vi "Toolbar Faacade.vi"(0 "Data In":T5, 2 "Display State In":T2={"Buttons Displayed"=0, "Button States"=[], "Button Size"=0, "Button Style"=enum."Classic", "Active Button"=0, "Force Regen?"=FALSE, "Tip String Ref"=refnum}, 3 "Container State":T4) -> (6 "Data Out":T5, 7 "Display State Out":T2={"Buttons Displayed"=0, "Button States"=[], "Button Size"=0, "Button Style"=enum."Classic", "Active Button"=0, "Force Regen?"=FALSE, "Tip String Ref"=refnum}, 8 "Action":T1)   [LabVIEW 2012, in "Toolbar.xctl"]
doc: "The business end of the XControl..."
uses:
  Toolbar.xctl
  Toolbar Data.ctl
  Button_Class/Type Defs/Button Events.ctl
  <vilib>/_xctls/Container State.ctl
  Toolbar State.ctl
  Button_Class/Button.lvclass
  Button_Class/Type Defs/Button Style.ctl
  <vilib>/_xctls/Action.ctl
  Button_Class/Type Defs/Button Status.ctl
  <vilib>/_xctls/XControlSupport.lvlib
panel:
  out "Display":picture[](array[picture])
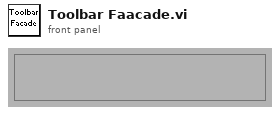
[diagram p1: front panel]
types:
  T1 = typedef "XControlSupport.lvlib/Action.ctl" = cluster{"Data Changed?":bool, "State Changed?":bool, "Action Name":string}
  T2 = typedef "Toolbar.xctl/Toolbar State.ctl" = cluster{"Buttons Displayed":i32, "Button States":refnum<class "Button.lvclass">[], "Button Size":i32, "Button Style":T3, "Active Button":i32, "Force Regen?":bool, "Tip String Ref":refnum<vi>}
  T3 = typedef "Button.lvclass/Button Style.ctl" = enum16{"System", "Modern", "Classic", "Rounded", "Silver", "Ni Theme", "Metallic"}
  T4 = typedef "XControlSupport.lvlib/Container State.ctl" = cluster{"Indicator?":bool, "Run Mode?":bool, " Refnum":refnum<vi>}
  T5 = typedef "Toolbar.xctl/Toolbar Data.ctl" = cluster{"Index":i32, "Type":T6}
  T6 = typedef "Button.lvclass/Button Events.ctl" = enum16{"Click", "Latch", "Unlatch"}
  T7 = enum16{"NoButton", "Left Button", "Right Button", "Middle Button"}
  T8 = typedef "Button.lvclass/Button Status.ctl" = enum16{"Off", "Hover", "On", "Disabled"}
  T9 = typedef "LVPoint32TypeDef.ctl" = cluster{"Horizontal":i32, "Vertical":i32}
  T10 = typedef "LVRectTypeDef.ctl" = cluster{"Left":i16, "Top":i16, "Right":i16, "Bottom":i16}
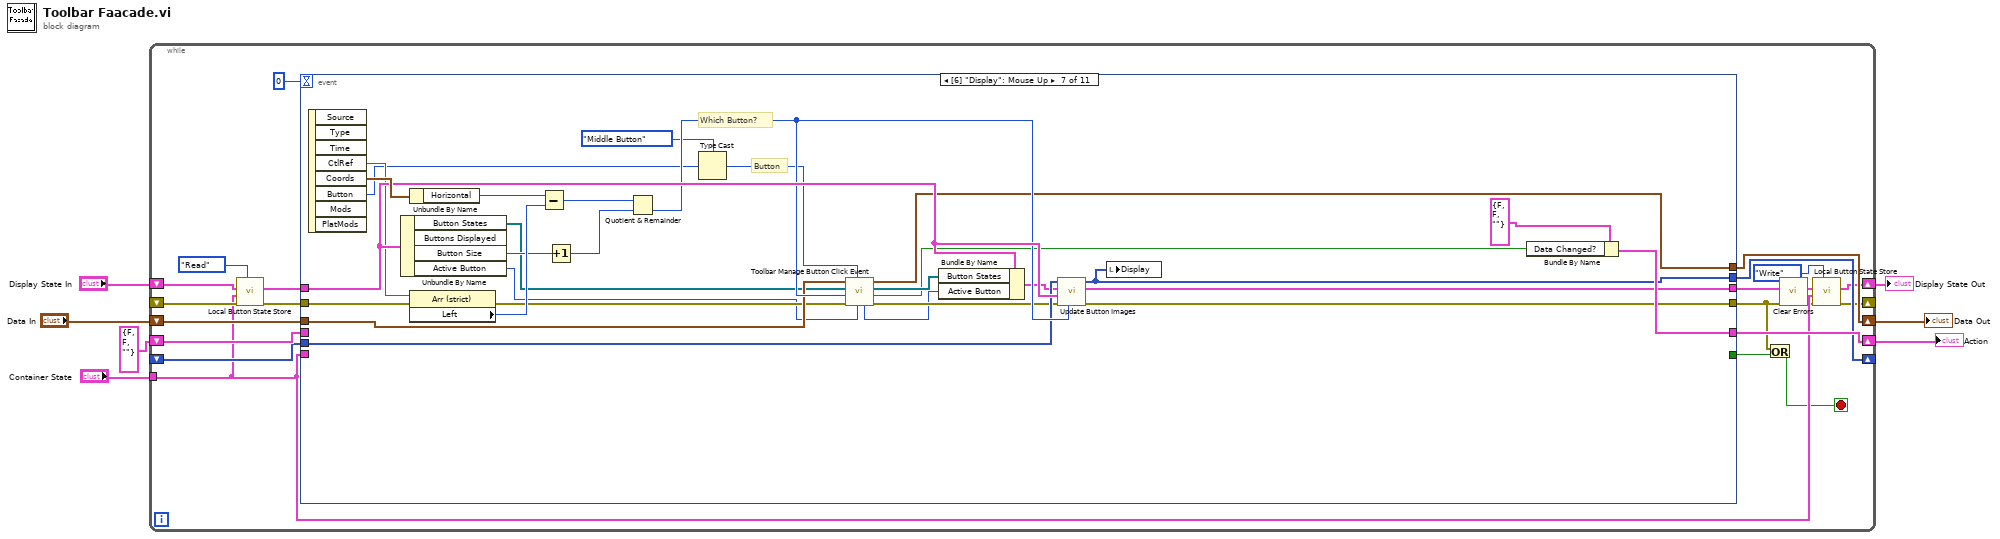
[diagram p0: block diagram]
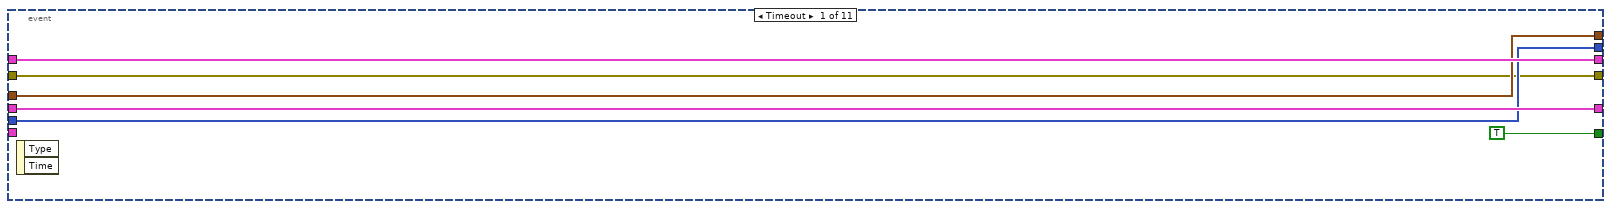
[diagram p2: hidden frame]
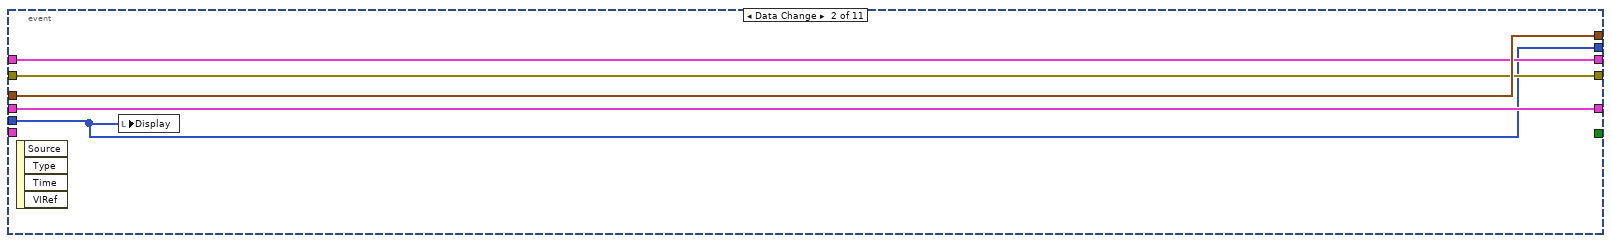
[diagram p3: hidden frame]
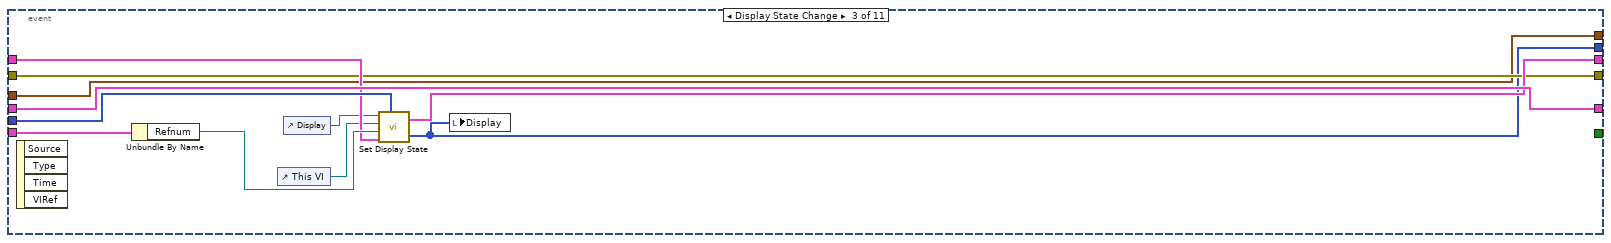
[diagram p4: hidden frame]
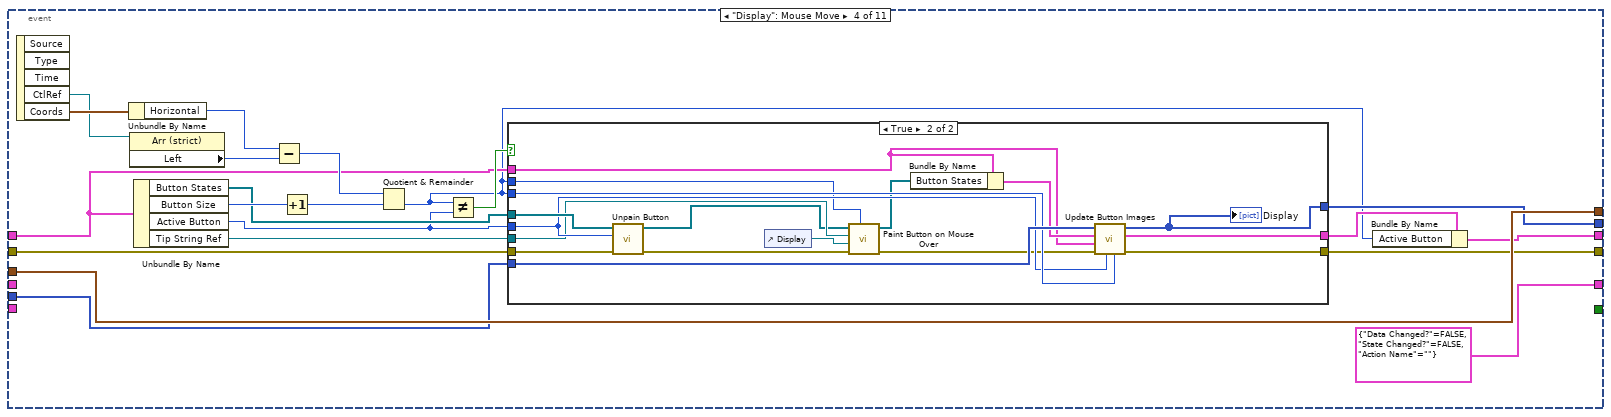
[diagram p5: hidden frame]
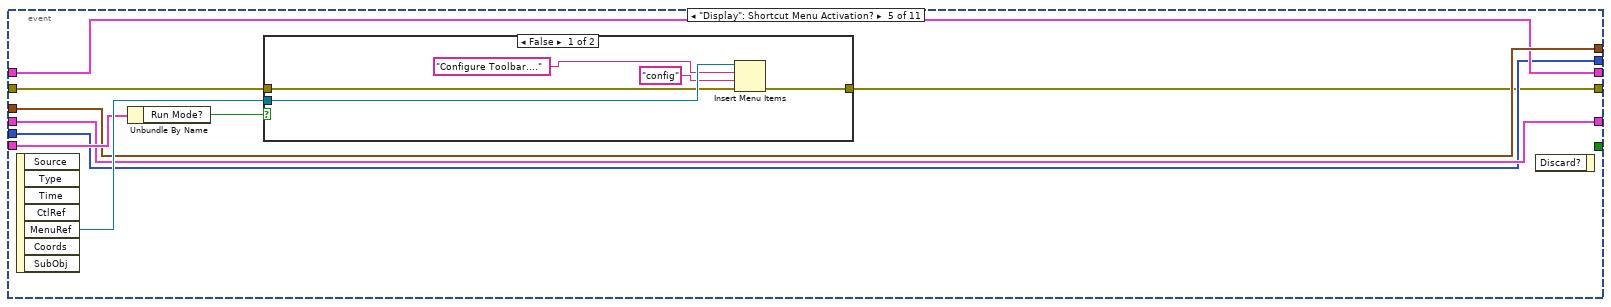
[diagram p7: hidden frame]
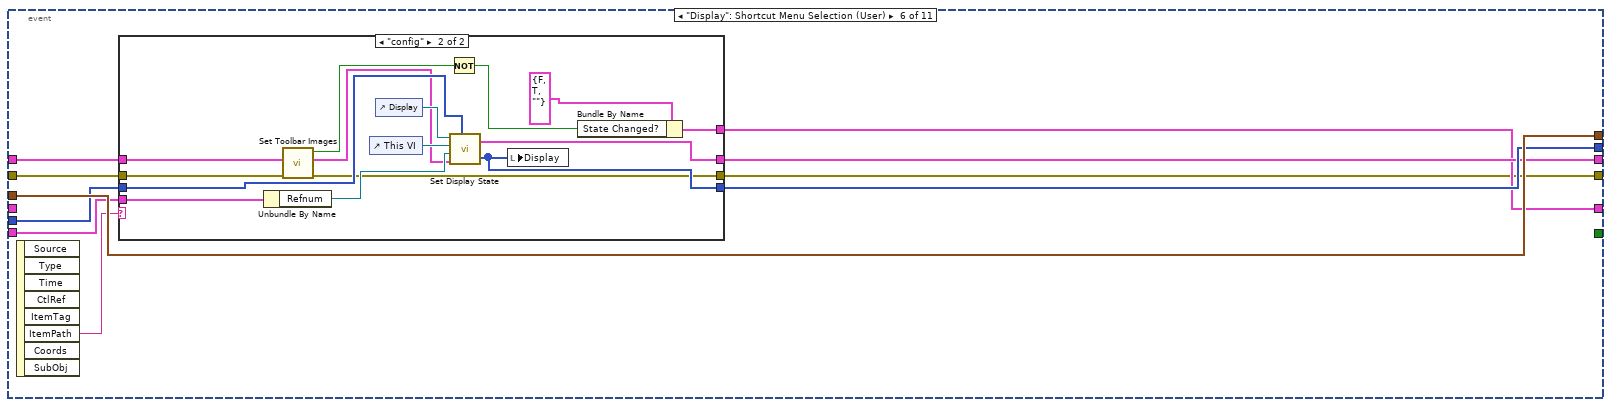
[diagram p9: hidden frame]
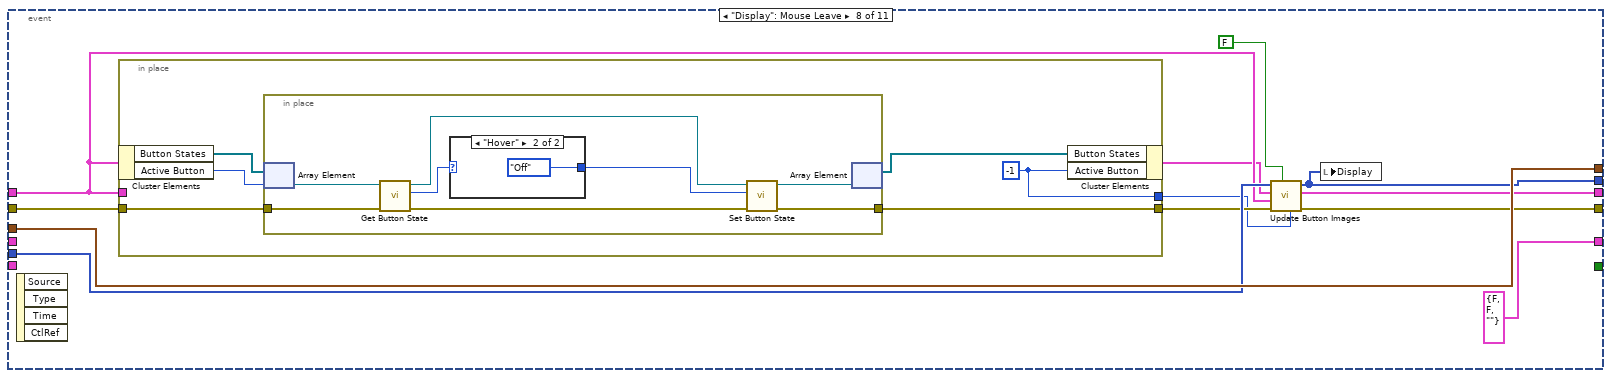
[diagram p11: hidden frame]
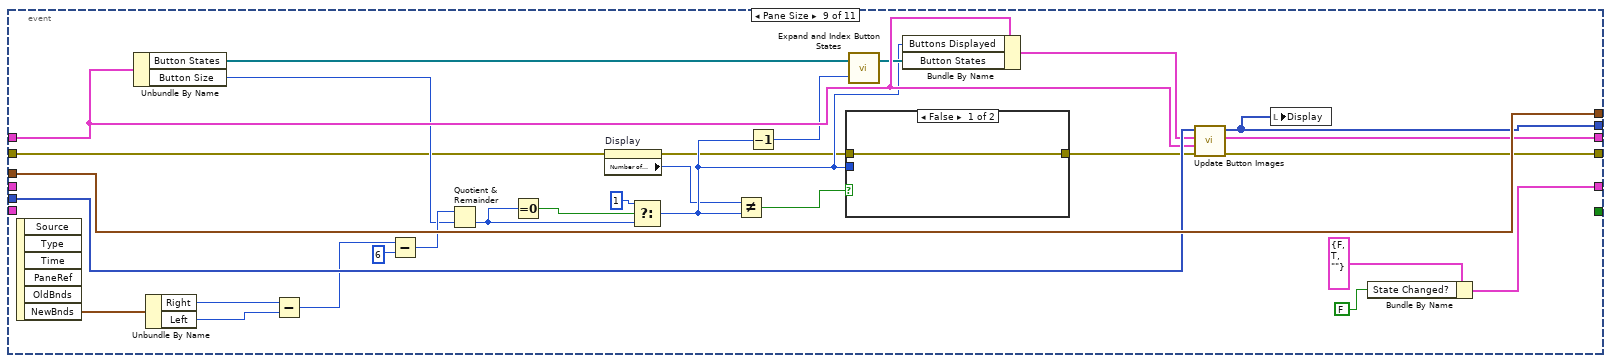
[diagram p13: hidden frame]
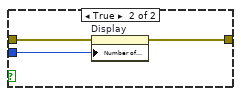
[diagram p14: hidden frame]
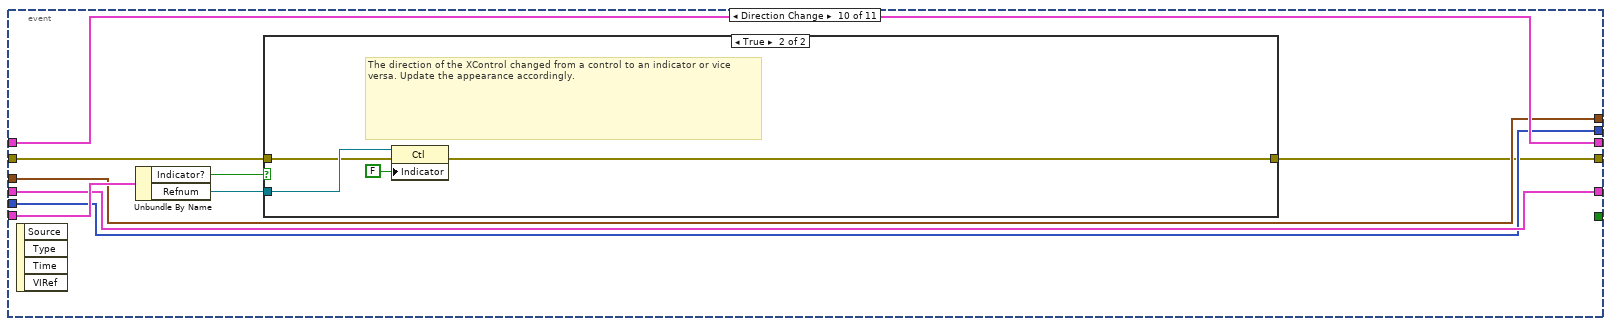
[diagram p15: hidden frame]
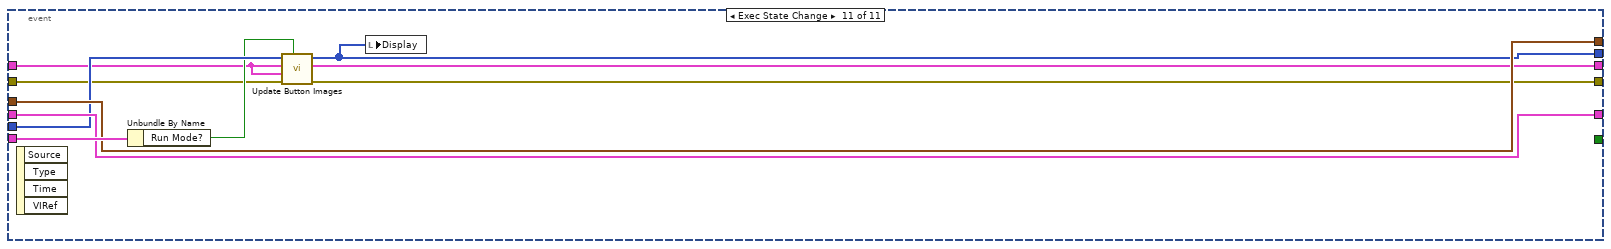
[diagram p17: hidden frame]
diagram:
  n1 = while {
    shift-right: [w11] -> w4
    shift-left: "Display State In" -> [w15]
    tunnel: "Container State" -> [w13]
    shift-right: [w25] -> w7
    shift-left: "Data In" -> [w26]
    shift-right: [w23] -> w2
    shift-left: T1 {"Data Changed?"=FALSE, "State Changed?"=FALSE, "Action Name"=""} ("Action") -> [w24]
    shift-right: [w22] -> _
    shift-left: _ -> [w21]
    shift-right: [w18] -> _
    shift-left: _ -> [w17]
    stop <- w10 stop-if-true
    n2 = call "Local Button State Store.vi"("Operation"=enum16{"Read", "Write"}."Read", "error in (no error)"=w17, "Container State"=w13, "Display State In"=w15) -> ("error out"=w16:errorcluster, "Display State Out"=w12:T2)  [unwired: 6 out]
    n3 = event shown="[6] \"Display\": Mouse Up" {
      selector: _ -> [_ _ _ _ _ _ _ _ _ _ _]
      dyn-events: _ -> [_ _ _ _ _ _ _ _ _ _ _]
      timeout: 0 -> [_ _ _ _ _ _ _ _ _ _ _]
      tunnel: w12 -> [w32 w38 w46 w55 w96 w115 w160 w167 w209 w232 w242]
      tunnel: [w32 w38 w43 w54 w96 w112 w155 w172 w207 w232 w241] -> w14
      tunnel: [TRUE _ _ _ _ _ _ _ _ _ _] -> w28
      tunnel: w13 -> [_ _ w48 _ w99 w111 _ _ _ w233 w248]
      tunnel: w26 -> [w31 w39 w41 w68 w97 w116 w153 w174 w215 w231 w247]
      tunnel: [w31 w39 w41 w68 w97 w116 w152 w174 w215 w231 w247] -> w25
      tunnel: [w33 w37 w50 T1 {"Data Changed?"=FALSE, "State Changed?"=FALSE, "Action Name"=""} ("Action") w95 w110 w163 T1 {"Data Changed?"=FALSE, "State Changed?"=FALSE, "Action Name"=""} ("Action") w200 w230 w246] -> w23
      tunnel: w24 -> [w33 w37 w50 _ w95 _ _ _ _ w230 w246]
      tunnel: [w30 w35 w40 w64 w94 w113 w151 w164 w193 w229 w244] -> w22
      tunnel: w21 -> [w30 w35 w49 w63 w94 w114 w150 w173 w213 w229 w245]
      tunnel: [w29 w36 w42 w59 w93 w108 w145 w169 w197 w225 w239] -> w9
      tunnel: w16 -> [w29 w36 w42 w58 w92 w109 w144 w171 w194 w226 w240]
      event Timeout {
        n4 = event-data() -> ()  [unwired: 3 out]
      }
      event Data Change {
        n5 = event-data() -> ()  [unwired: 5 out]
        n6 = local write "Display"(w35) -> ()
      }
      event Display State Change {
        n7 = event-data() -> ()  [unwired: 5 out]
        n8 = Unbundle By Name(w48) -> ("Refnum"=w47:refnum<vi>)
        n9 = control-ref of="This VI"() -> (w45:refnum<vi>)
        n10 = control-ref of="Display"() -> (w44:refnum<vi>)
        n11 = call "Set Display State.vi"("Picture Array Refnum"=w44, "Facade Vi Refnum"=w45, "Container Refnum"=w47, "Display State In"=w46, "Display"=w49) -> ("State Out"=w43:T2, "Images Out"=w40:picture[])
        n12 = local write "Display"(w40) -> ()
      }
      event "Display": Mouse Move {
        n13 = event-data() -> ("CtlRef"=w67:refnum<vi>, "Coords"=w70:T9)  [unwired: 4 out]
        n14 = Unbundle By Name(w70) -> ("Horizontal"=w69:i32)
        n15 = property class="Arr (strict)"(reference=w67) -> ("Left"=w65:i32)  [unwired: 1 in, 2 out]
        n16 = Unbundle By Name(w55) -> ("Button States"=w57:refnum<class "Button.lvclass">[], "Button Size"=w61:i32, "Active Button"=w52:i32, "Tip String Ref"=w51:refnum<vi>)
        n17 = Subtract(x=w69, y=w65) -> (x-y=w66:i32)
        n18 = Increment(x=w61) -> (x+1=w60:i32)
        n19 = Quotient & Remainder(x=w66, y=w60) -> (floor(x/y)=w53:i32)  [unwired: 1 out]
        n20 = Not Equal?(x=w53, y=w52) -> (x != y?=w56:bool)
        n21 = case shown="True" w56 {
          tunnel: [w74 w80] -> w64
          tunnel: w63 -> [w74 w91]
          tunnel: w55 -> [w73 w79]
          tunnel: [w73 w89] -> w62
          tunnel: [w72 w75] -> w59
          tunnel: w58 -> [w72 w85]
          tunnel: w57 -> [_ w87]
          tunnel: w53 -> [_ w84]
          tunnel: w52 -> [_ w86]
          tunnel: w53 -> [_ w88]
          tunnel: w51 -> [_ w78]
          frame False {
          }
          frame True {
            n22 = call "Unpain Button.vi"("error in (no error)"=w85, "Old Button"=w86, "Button States in"=w87) -> ("error out"=w83:errorcluster, "Button States out"=w77:refnum<class "Button.lvclass">[])  [unwired: 7 in]
            n23 = control-ref of="Display"() -> (w76:refnum<vi>)
            n24 = call "Paint Button on Mouse Over.vi"("New Active Button"=w84, "error in (no error)"=w83, "Array in"=w76, "Tip String Ref"=w78, "Button States in"=w77) -> ("error out"=w81:errorcluster, "Button States out"=w82:refnum<class "Button.lvclass">[])  [unwired: 5 in]
            n25 = Bundle By Name(cluster=w79, "Button States"=w82) -> (w90:T2)
            n26 = call "Update Button Images.vi"("New Index"=w88, "Old Index"=w86, "error in (no error)"=w81, "Old State"=w79, "New State"=w90, "Images In"=w91) -> ("error out"=w75:errorcluster, "State Out"=w89:T2, "Images Out"=w80:picture[])  [unwired: 1 in, 2 out]
            "Display" <- w80
          }
        }
        n27 = Bundle By Name(cluster=w62, "Active Button"=w53) -> (w54:T2)
      }
      event "Display": Shortcut Menu Activation? {
        n28 = event-data() -> ("MenuRef"=w100:refnum<k9>)  [unwired: 7 out]
        n29 = Unbundle By Name(w99) -> ("Run Mode?"=w98:bool)
        n30 = case shown="False" w98 {
          tunnel: w100 -> [w105 _]
          tunnel: [w102 w106] -> w93
          tunnel: w92 -> [w101 w106]
          frame False {
            n31 = Insert Menu Items(6:w101, 7:"config" ("item tags"), 8:"Configure Toolbar....", 9:w105) -> (0:w102:errorcluster)  [unwired: 4 out]
          }
          frame True {
          }
        }
        n32 = event-data() -> ()  [unwired: 1 in, 2 out]
      }
      event "Display": Shortcut Menu Selection (User) {
        n33 = event-data() -> ("ItemPath"=w107:string)  [unwired: 8 out]
        n34 = case shown="\"config\"" w107 {
          tunnel: w115 -> [w119 w133]
          tunnel: w114 -> [w117 w125]
          tunnel: [w117 w126] -> w113
          tunnel: [w119 w130] -> w112
          tunnel: w111 -> [_ w129]
          tunnel: [_ w127] -> w110
          tunnel: w109 -> [w118 w124]
          tunnel: [w118 w123] -> w108
          frame "False", Default {
          }
          frame "config" {
            n35 = Unbundle By Name(w129) -> ("Refnum"=w128:refnum<vi>)
            n36 = call "Set Toolbar Images.vi"("error in (no error)"=w124, "State"=w133) -> ("error out"=w123:errorcluster, "State Out"=w120:T2, "Cancelled?"=w122:bool)  [unwired: 7 out]
            n37 = control-ref of="This VI"() -> (w132:refnum<vi>)
            n38 = control-ref of="Display"() -> (w131:refnum<vi>)
            n39 = Not(x=w122) -> (.not. x?=w121:bool)
            n40 = call "Set Display State.vi"("Picture Array Refnum"=w131, "Facade Vi Refnum"=w132, "Container Refnum"=w128, "Display State In"=w120, "Display"=w125) -> ("State Out"=w130:T2, "Images Out"=w126:picture[])
            n41 = local write "Display"(w126) -> ()
            n42 = Bundle By Name(cluster=T1 {"Data Changed?"=FALSE, "State Changed?"=TRUE, "Action Name"=""} ("Action"), "State Changed?"=w121) -> (w127:T1)
          }
        }
      }
      event "Display": Mouse Up {
        # "Which Button?"
        # "Button"
        n43 = event-data() -> ("CtlRef"=w158:refnum<vi>, "Coords"=w162:T9, "Button"=w154:u16)  [unwired: 6 out]
        n44 = Unbundle By Name(w160) -> ("Button States"=w141:refnum<class "Button.lvclass">[], "Button Size"=w149:i32, "Active Button"=w142:i32)  [unwired: 1 out]
        n45 = Unbundle By Name(w162) -> ("Horizontal"=w161:i32)
        n46 = property class="Arr (strict)"(reference=w158, error in=w144) -> (error out=w143:errorcluster, "Left"=w156:i32)  [unwired: 1 out]
        n47 = Subtract(x=w161, y=w156) -> (x-y=w157:i32)
        n48 = Increment(x=w149) -> (x+1=w148:i32)
        n49 = Quotient & Remainder(x=w157, y=w148) -> (floor(x/y)=w159:i32)  [unwired: 1 out]
        n50 = Type Cast(type=T7."Middle Button", x=w154) -> (*(type *) &x=w147:T7)
        n51 = call "Toolbar Manage Button Click Event.vi"("Index In"=w142, "Button"=w147, "error in (no Error)"=w143, "Button Index"=w159, "Button States In"=w141, "Data In"=w153) -> ("error out"=w138:errorcluster, "Data Changed ?"=w136:bool, "Button States Out"=w137:refnum<class "Button.lvclass">[], "Data Out"=w152:T5, "Index Out"=w135:i32)  [unwired: 1 out]
        n52 = Bundle By Name(cluster=w160, "Button States"=w137, "Active Button"=w135) -> (w139:T2)
        n53 = call "Update Button Images.vi"("Old Index"=w159, "error in (no error)"=w138, "Old State"=w160, "New State"=w139, "Images In"=w150) -> ("error out"=w145:errorcluster, "State Out"=w155:T2, "Images Out"=w151:picture[])  [unwired: 2 in, 2 out]
        n54 = local write "Display"(w151) -> ()
        n55 = Bundle By Name(cluster=T1 {"Data Changed?"=FALSE, "State Changed?"=FALSE, "Action Name"=""} ("Action"), "Data Changed?"=w136) -> (w163:T1)
      }
      event "Display": Mouse Leave {
        n56 = event-data() -> ()  [unwired: 5 out]
        n57 = in-place {
          in-place-border: w167 -> [_]
          in-place-border: w171 -> [w181]
          in-place-border: [w180] -> w170
          in-place-border: [w176] -> w168
          w176 = -1
          n58 = in-place-cluster #1(w167) -> ("Button States"=w179:refnum<class "Button.lvclass">[], "Active Button"=w178:i32)
          n59 = in-place {
            in-place-border: w181 -> [w189]
            in-place-border: [w188] -> w180
            n60 = in-place-array #2(w179, w178) -> (w183:refnum<class "Button.lvclass">)
            n61 = call-dynamic "Get Button State.vi"("error in (no error)"=w189, "Button in"=w183) -> ("error out"=w184:errorcluster, "State"=w185:T8, "Button out"=w186:refnum<class "Button.lvclass">)  [unwired: 7 out]
            n62 = case shown="\"Hover\"" w185 {
              selector: w185 -> [w190 _]
              tunnel: [w190 Button_Status."Off" ("State")] -> w187
              frame "Off", Default {
              }
              frame "Hover" {
              }
            }
            n63 = call-dynamic "Set Button State.vi"("error in (no error)"=w184, "State"=w187, "Button in"=w186) -> ("error out"=w188:errorcluster, "Button out"=w182:refnum<class "Button.lvclass">)  [unwired: 7 out]
            n64 = in-place-array #2(w182) -> (w177:refnum<class "Button.lvclass">[])  [unwired: 1 out]
          }
          n65 = in-place-cluster #1("Button States"=w177, "Active Button"=w176) -> (w166:T2)
        }
        n66 = call "Update Button Images.vi"("New Index"=w168, "Force Regen"=FALSE, "error in (no error)"=w170, "Old State"=w167, "New State"=w166, "Images In"=w173) -> ("error out"=w169:errorcluster, "State Out"=w172:T2, "Images Out"=w164:picture[])  [unwired: 1 in, 2 out]
        n67 = local write "Display"(w164) -> ()
      }
      event Pane Size {
        n68 = event-data() -> ("NewBnds"=w201:T10)  [unwired: 6 out]
        n69 = Unbundle By Name(w209) -> ("Button States"=w192:refnum<class "Button.lvclass">[], "Button Size"=w206:i32)
        n70 = Unbundle By Name(w201) -> ("Right"=w220:i16, "Left"=w219:i16)
        n71 = Subtract(x=w220, y=w219) -> (x-y=w211:i16)
        n72 = Subtract(x=w211, y=i16 6) -> (x-y=w212:i16)
        n73 = Quotient & Remainder(x=w212, y=w206) -> (floor(x/y)=w218:i32)  [unwired: 1 out]
        n74 = Equal To 0?(x=w218) -> (x = 0?=w214:bool)
        n75 = property on="Display" class="Arr (strict)"(error in=w194) -> (error out=w195:errorcluster, "Number of Columns"=w202:u32)  [unwired: 1 in, 1 out]
        n76 = Select(t=i16 1, s=w214, f=w218) -> (s? t:f=w203:i32)
        n77 = Not Equal?(x=w202, y=w203) -> (x != y?=w199:bool)
        n78 = Decrement(x=w203) -> (x-1=w204:i32)
        n79 = case shown="False" w199 {
          tunnel: w203 -> [_ w224]
          tunnel: [w221 w223] -> w196
          tunnel: w195 -> [w221 w222]
          frame False {
          }
          frame True {
            n80 = property on="Display" class="Arr (strict)"(error in=w222, "Number of Columns"=w224) -> (error out=w223:errorcluster)  [unwired: 1 in, 1 out]
          }
        }
        n81 = call "Expand and Index Button States.vi"("Button Index"=w204, "Button States"=w192) -> ("Button States Out"=w205:refnum<class "Button.lvclass">[])  [unwired: 1 out]
        n82 = Bundle By Name(cluster=w209, "Buttons Displayed"=w203, "Button States"=w205) -> (w208:T2)
        n83 = call "Update Button Images.vi"("error in (no error)"=w196, "Old State"=w209, "New State"=w208, "Images In"=w213) -> ("error out"=w197:errorcluster, "State Out"=w207:T2, "Images Out"=w193:picture[])  [unwired: 3 in, 2 out]
        n84 = local write "Display"(w193) -> ()
        n85 = Bundle By Name(cluster=T1 {"Data Changed?"=FALSE, "State Changed?"=TRUE, "Action Name"=""} ("Action"), "State Changed?"=FALSE) -> (w200:T1)
      }
      event Direction Change {
        n86 = event-data() -> ()  [unwired: 5 out]
        n87 = Unbundle By Name(w233) -> ("Indicator?"=w227:bool, "Refnum"=w228:refnum<vi>)
        n88 = case shown="True" w227 {
          tunnel: w228 -> [_ w238]
          tunnel: w226 -> [w234 w236]
          tunnel: [w234 w235] -> w225
          frame False {
          }
          frame True {
            # "The direction of the XControl changed from a control to an indicator or vice versa. Update the appearance accordingly."
            n89 = property class="Ctl"(reference=w238, error in=w236, "Indicator"=FALSE) -> (error out=w235:errorcluster)  [unwired: 1 out]
          }
        }
      }
      event Exec State Change {
        n90 = event-data() -> ()  [unwired: 5 out]
        n91 = Unbundle By Name(w248) -> ("Run Mode?"=w243:bool)
        n92 = call "Update Button Images.vi"("Force Regen"=w243, "error in (no error)"=w240, "Old State"=w242, "New State"=w242, "Images In"=w245) -> ("error out"=w239:errorcluster, "State Out"=w241:T2, "Images Out"=w244:picture[])  [unwired: 2 in, 2 out]
        n93 = local write "Display"(w244) -> ()
      }
    }
    n94 = Or(x=w9, y=w28) -> (x .or. y?=w10:bool)
    n95 = call <vilib>:"Clear Errors.vi"("error in (no error)"=w9) -> ("error out"=w8:errorcluster)  [unwired: 6 in]
    n96 = call "Local Button State Store.vi"("Operation"=enum16{"Read", "Write"}."Write", "error in (no error)"=w8, "Container State"=w13, "Display State In"=w14) -> ("error out"=w18:errorcluster, "Display State Out"=w11:T2)  [unwired: 1 in, 5 out]
  }
  "Display State Out" <- w4
  "Data Out" <- w7
  "Action" <- w2
